vi "Cleanup Session.vi"(8 "error in":errorcluster, 11 "Plugin in":refnum<class "Nominal-Streamer.lvclass">) -> (0 "error out":errorcluster, 3 "Plugin out":refnum<class "Nominal-Streamer.lvclass">)   [LabVIEW 2020, in "Nominal-Streamer.lvlib" / "Nominal-Streamer.lvclass"]
uses:
  Nominal-Streamer.lvclass
  Nominal-Streamer.lvclass/Nominal-Streamer.ctl
  async queue data.ctl
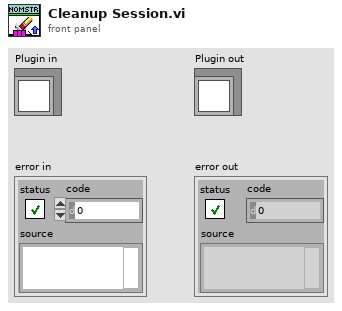
[diagram p1: front panel]
types:
  T1 = typedef "Nominal-Streamer.lvlib/Nominal-Streamer.lvclass/async queue data.ctl" = cluster{"data values":waveform(dbl)[], "data names":string[]}
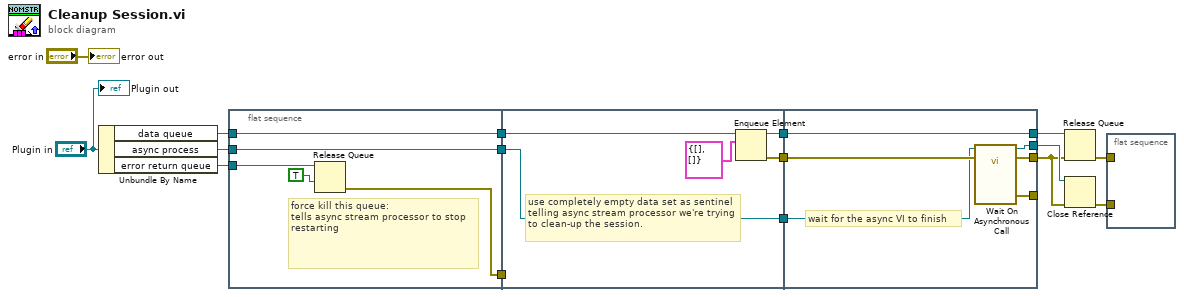
[diagram p0: block diagram]
diagram:
  n1 = Unbundle By Name("Plugin in") -> ("data queue"=w16:refnum<queue>, "async process"=w3:refnum<vi>, "error return queue"=w9:refnum<queue>)
  n2 = flat-sequence {
    tunnel: w16 -> [w21]
    tunnel: [w21] -> w11
    tunnel: [w18] -> w10
    tunnel: w9 -> [w20]
    tunnel: w3 -> [w17]
    tunnel: [w17] -> w2
    tunnel: w11 -> [w26]
    tunnel: w10 -> [_]
    tunnel: [w25] -> w8
    tunnel: [w23] -> w7
    tunnel: w2 -> [w22]
    tunnel: [w22] -> w1
    tunnel: [w32] -> w15
    tunnel: w8 -> [w32]
    tunnel: w7 -> [w31]
    tunnel: [w30] -> w6
    tunnel: [w29] -> w5
    tunnel: [w28] -> _
    tunnel: w1 -> [w27]
    frame #0 {
      # "force kill this queue:\ntells async stream processor to stop restarting"
      n3 = Release Queue(queue=w20, force destroy? (F)=TRUE) -> (error out=w18:errorcluster)  [unwired: 1 in, 2 out]
    }
    frame #1 {
      # "use completely empty data set as sentinel telling async stream processor we're trying to clean-up the session."
      n4 = Enqueue Element(queue=w26, element=T1 {"data values"=[], "data names"=[]}) -> (queue out=w25:refnum<queue>, error out=w23:errorcluster)  [unwired: 2 in, 1 out]
    }
    frame #2 {
      # "wait for the async VI to finish"
      n5 = call-by-ref "Wait On Asynchronous Call"(reference=w27, error in=w31) -> (reference out=w30:refnum<vi>, error out=w29:errorcluster, "last error"=w28:errorcluster)  [unwired: 11 in]
    }
  }
  n6 = Release Queue(queue=w15, error in (no error)=w5) -> (error out=w13:errorcluster)  [unwired: 1 in, 2 out]
  n7 = Close Reference(reference=w6, error in (no error)=w5) -> (error out=w12:errorcluster)
  n8 = flat-sequence {
    tunnel: w13 -> [_]
    tunnel: w12 -> [_]
    frame #0 {
    }
  }
  "error out" <- "error in"
  "Plugin out" <- "Plugin in"
